vi "Parse Result Key.vi"(8 "error in (no error)":errorcluster, 9 "Ref Channel":i32, 10 "AI Channel":i32, 11 "Datatype":T1) -> (0 "error out":errorcluster, 2 "Label":string, 3 "Key":string)   [LabVIEW 2019, in "Instrument.Lockin.lvlib" / "Instrument.Lockin.lvclass"]
uses:
  Instrument.Lockin.lvclass
  Typedefs/Results Type--Enum.ctl
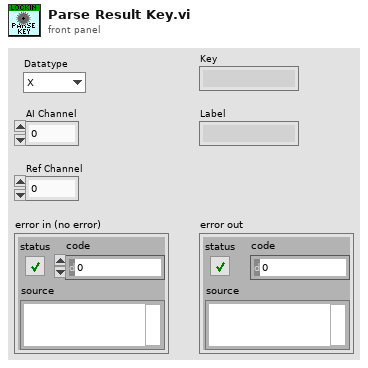
[diagram p1: front panel]
types:
  T1 = typedef "Instrument.Lockin.lvlib/Instrument.Lockin.lvclass/Results Type--Enum.ctl" = enum16{"X", "Y", "R", "Theta", "Mean"}
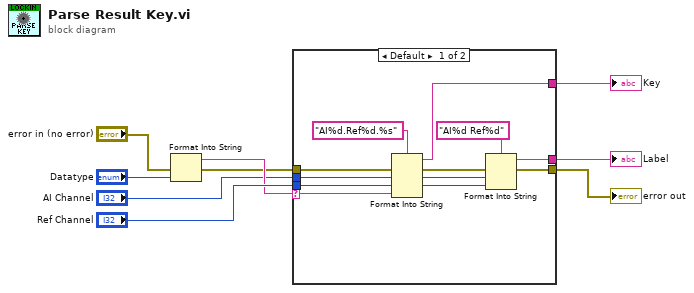
[diagram p0: block diagram]
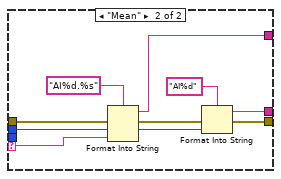
[diagram p2: hidden frame]
diagram:
  n1 = Format Into String(error in="error in (no error)", "Datatype") -> (resulting string=w5:string, error out=w2:errorcluster)  [unwired: 2 in]
  n2 = case shown="Default" w5 {
    selector: w5 -> [w10 w20]
    tunnel: "Ref Channel" -> [w11 _]
    tunnel: "AI Channel" -> [w19 w28]
    tunnel: [w18 w27] -> w9
    tunnel: w2 -> [w17 w26]
    tunnel: [w15 w24] -> w8
    tunnel: [w13 w22] -> w7
    frame Default {
      n3 = Format Into String(format string="AI%d.Ref%d.%s", error in=w17, w19, w11, w10) -> (resulting string=w13:string, error out=w16:errorcluster)  [unwired: 1 in]
      n4 = Format Into String(format string="AI%d Ref%d", error in=w16, w19, w11) -> (resulting string=w15:string, error out=w18:errorcluster)  [unwired: 1 in]
    }
    frame "Mean" {
      n5 = Format Into String(format string="AI%d.%s", error in=w26, w28, w20) -> (resulting string=w22:string, error out=w25:errorcluster)  [unwired: 1 in]
      n6 = Format Into String(format string="AI%d", error in=w25, w28) -> (resulting string=w24:string, error out=w27:errorcluster)  [unwired: 1 in]
    }
  }
  "error out" <- w9
  "Label" <- w8
  "Key" <- w7
